vi "FX232_485_RRRSTT.vi"(5 "延时":u8 max=150 step=10, 7 "PLC站号":u8=1, 8 "error in (no error)":errorcluster caption="错误输入（无错误）", 9 "值":string, 10 "命令":string(combo), 11 "Port":refnum<visa-resource-name>) -> (0 "error out":errorcluster caption="错误输出", 1 "Value":string, 2 "Buff":string, 3 "PortOut":refnum<visa-resource-name>)   [LabVIEW 2025]
uses:
  <vilib>/Utility/error.llb/Trim Whitespace One-Sided.vi
panel:
  out "连接的字符串":string
  # "X,Y,D,S,M"
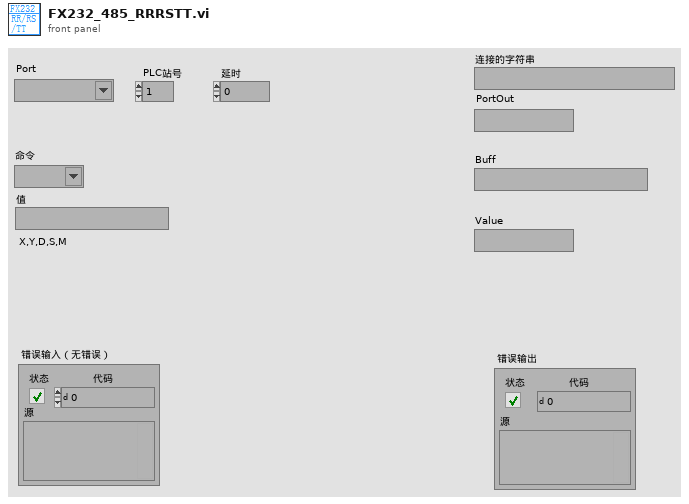
[diagram p1: front panel]
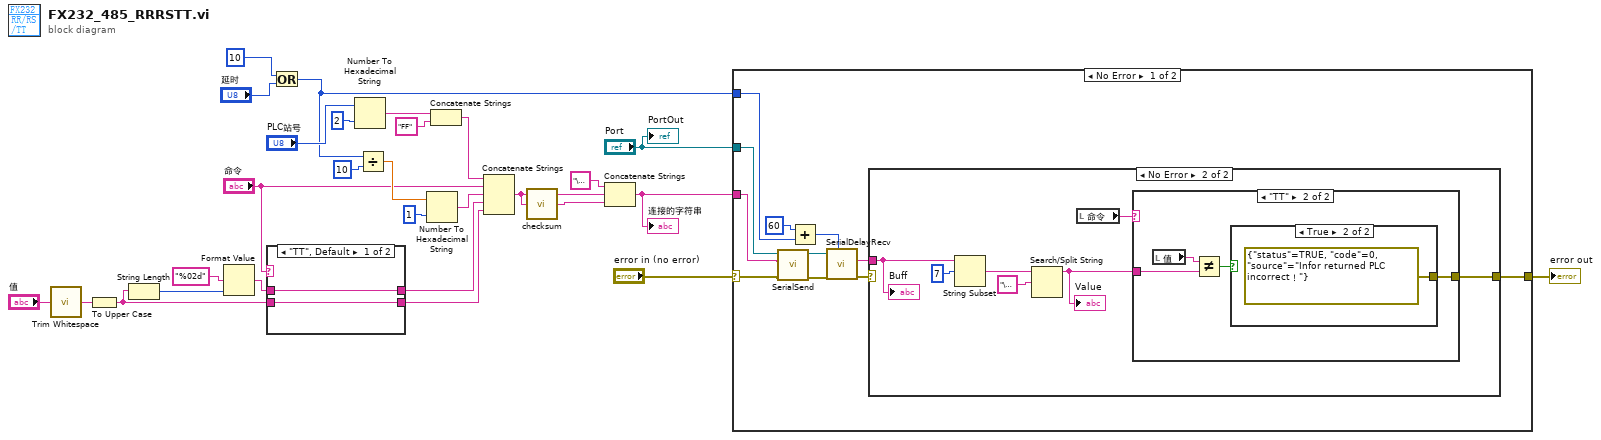
[diagram p0: block diagram]
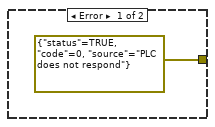
[diagram p3: hidden frame]
diagram:
  n1 = call <vilib>:"Trim Whitespace.vi"("string"="值") -> ("trimmed string"=w27:string)  [unwired: 1 in]
  n2 = To Upper Case(1:w27) -> (0:w10:string)
  n3 = String Length(string=w10) -> (length=w11:i32)
  n4 = Format Value(format string="%02d" ("格式字符串"), value (0)=w11) -> (output string=w13:string)  [unwired: 1 in]
  n5 = case shown="\"TT\", Default" "命令" {
    tunnel: w13 -> [w30 _]
    tunnel: [w30 _] -> w12
    tunnel: [w29 _] -> w6
    tunnel: w10 -> [w29 _]
    frame "TT", Default {
    }
    frame "PC", "RR", "RS" {
    }
  }
  n6 = Or(x=u8 10, y="延时") -> (x .or. y?=w2:u8)
  n7 = Number To Hexadecimal String(1:i16 2 ("宽度(-)"), 2:"PLC站号") -> (0:w18:string)
  n8 = Divide(x=w2, y=10) -> (x/y=w22:dbl)
  n9 = Number To Hexadecimal String(1:i16 1 ("宽度(-)"), 2:w22) -> (0:w17:string)
  n10 = Concatenate Strings(w18, "FF" ("字符串")) -> (w15:string)
  n11 = Concatenate Strings(w15, "命令", w17, w12, w6) -> (w5:string)
  n12 = call "checksum.vi"("buff"=w5) -> ("checksum"=w4:string)  [unwired: 4 in]
  n13 = Concatenate Strings("\u0005" ("字符串"), w5, w4) -> (w20:string)
  "连接的字符串" <- w20
  n14 = case shown="No Error" "error in (no error)" {
    selector: "error in (no error)" -> [w33 w55]
    tunnel: w20 -> [w34 _]
    tunnel: "Port" -> [w35 _]
    tunnel: [w41 w55] -> w26
    tunnel: w2 -> [w40 _]
    frame No Error {
      n15 = call "SerialSend.vi"("error in (no error)"=w33, "SendData"=w34, "PORT"=w35) -> ("error out"=w32:errorcluster, "PORT out"=w31:refnum<visa-resource-name>)  [unwired: 6 in, 1 out]
      n16 = Add(x=u32 60 ("等待时间（毫秒）"), y=w40) -> (x+y=w36:u32)
      n17 = call "SerialDelayRecv.vi"("Timeout"=w36, "error in (no error)"=w32, "Port"=w31) -> ("error out"=w38:errorcluster, "Buff"=w37:string)  [unwired: 6 in, 1 out]
      n18 = case shown="No Error" w38 {
        tunnel: [errorcluster {"status"=TRUE, "code"=0, "source"="PLC does not respond"} ("错误常量") w44] -> w41
        tunnel: w37 -> [_ w43]
        frame Error {
        }
        frame No Error {
          n19 = String Subset(string=w43, offset (0)=7 ("长度（剩余）")) -> (substring=w48:string)  [unwired: 1 in]
          n20 = Search/Split String(string=w48, search string/char (-)="\u0003") -> (substring before match=w45:string)  [unwired: 1 in, 2 out]
          "Value" <- w45
          n21 = local read "命令"() -> (w46:string)
          n22 = case shown="\"TT\"" w46 {
            tunnel: w45 -> [_ w52]
            tunnel: [_ w50] -> w44
            frame "假", Default {
            }
            frame "TT" {
              n23 = local read "值"() -> (w53:string)
              n24 = Not Equal?(x=w53, y=w52) -> (x != y?=w51:bool)
              n25 = case shown="True" w51 {
                tunnel: [_ errorcluster {"status"=TRUE, "code"=0, "source"="Infor returned PLC incorrect！"} ("错误常量")] -> w50
                frame False {
                }
                frame True {
                }
              }
            }
          }
          "Buff" <- w43
        }
      }
    }
    frame Error {
    }
  }
  "error out" <- w26
  "PortOut" <- "Port"
